vi "set Starting and Num RB.vi"(8 "error in (no error)":errorcluster, 10 "RB Setting Param":T1, 11 "NR in":refnum<class "NR.lvclass">) -> (0 "error out":errorcluster, 3 "NR out":refnum<class "NR.lvclass">)   [LabVIEW 2023, in "ANRITSU Call Box.lvlib" / "NR.lvclass"]
uses:
  NR.lvclass
  NR.lvclass/NR.ctl
  Type Definition/NR RB Setting Params.ctl
  ANRITSU Call Box.lvlib
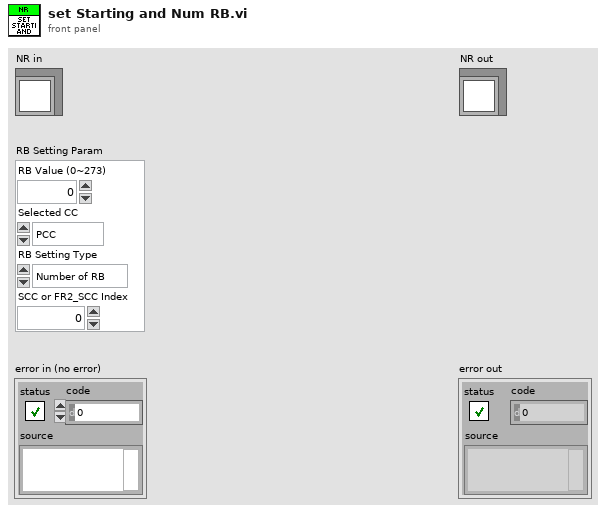
[diagram p1: front panel]
types:
  T1 = typedef "ANRITSU Call Box.lvlib/NR RB Setting Params.ctl" = cluster{"RB Value (0~273)":i32, "Selected CC":enum16{"PCC", "SCC", "FR2_PCC", "FR2_SCC"}, "RB Setting Type":enum16{"Number of RB", "Starting RB"}, "SCC or FR2_SCC Index":u32}
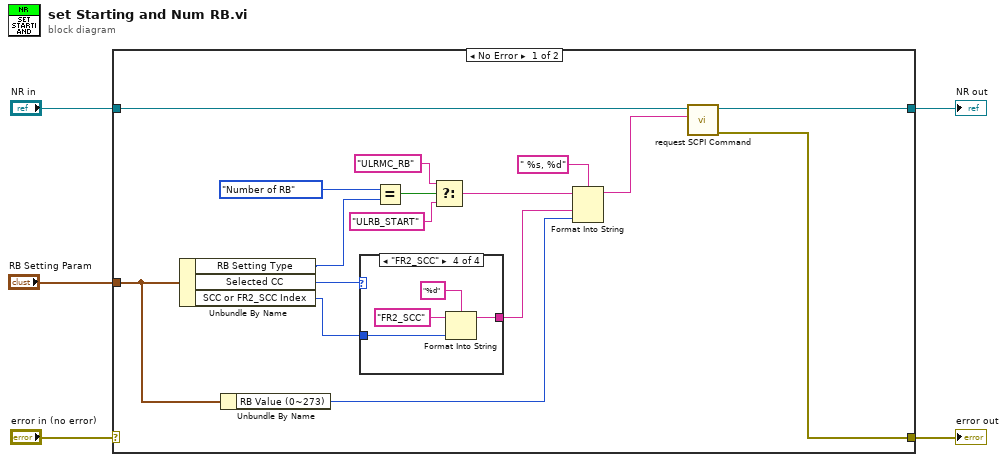
[diagram p0: block diagram]
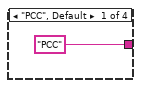
[diagram p2: hidden frame]
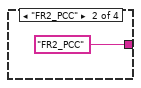
[diagram p3: hidden frame]
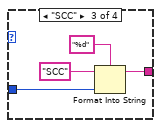
[diagram p4: hidden frame]
diagram:
  n1 = case shown="No Error" "error in (no error)" {
    selector: "error in (no error)" -> [_ w33]
    tunnel: [w19 w33] -> w2
    tunnel: [w20 w32] -> w4
    tunnel: "NR in" -> [w21 w32]
    tunnel: "RB Setting Param" -> [w16 _]
    frame No Error {
      n2 = Unbundle By Name(w16) -> ("RB Setting Type"=w11:enum16{"Number of RB", "Starting RB"}, "Selected CC"=w18:enum16{"PCC", "SCC", "FR2_PCC", "FR2_SCC"}, "SCC or FR2_SCC Index"=w17:u32)
      n3 = Unbundle By Name(w16) -> ("RB Value (0~273)"=w7:i32)
      n4 = case shown="\"FR2_SCC\"" w18 {
        tunnel: ["PCC" "FR2_PCC" w25 w29] -> w8
        tunnel: w17 -> [_ _ w24 w28]
        frame "PCC", Default {
        }
        frame "FR2_PCC" {
        }
        frame "SCC" {
          n5 = Format Into String(format string="%d", initial string="SCC", w24) -> (resulting string=w25:string)  [unwired: 1 in, 1 out]
        }
        frame "FR2_SCC" {
          n6 = Format Into String(format string="%d", initial string="FR2_SCC", w28) -> (resulting string=w29:string)  [unwired: 1 in, 1 out]
        }
      }
      n7 = Equal?(x=enum16{"Number of RB", "Starting RB"}."Number of RB", y=w11) -> (x = y?=w14:bool)
      n8 = Select(t="ULRMC_RB" ("format string"), s=w14, f="ULRB_START" ("format string")) -> (s? t:f=w9:string)
      n9 = Format Into String(format string=" %s, %d", initial string=w9, w8, w7) -> (resulting string=w6:string)  [unwired: 1 in, 1 out]
      n10 = call "request SCPI Command.vi"("SCPI Command"=w6, "NR in"=w21) -> ("error out"=w19:errorcluster, "NR out"=w20:refnum<class "NR.lvclass">)  [unwired: 8 in]
    }
    frame Error {
    }
  }
  "error out" <- w2
  "NR out" <- w4
